vi "Connect.vi"(8 "error in (no error)":errorcluster caption="에러 입력(에러 없음)", 9 "원격 포트 또는 서비스 이름":u16, 10 "주소":string, 11 "RF Filter Box 입력":refnum<class "RF Filter Box.lvclass">) -> (0 "error out":errorcluster caption="에러 출력", 2 "Connected?":bool, 3 "RF Filter Box 출력":refnum<class "RF Filter Box.lvclass">)   [LabVIEW 2023, in "RF Switch Box.lvlib" / "RF Filter Box.lvclass"]
uses:
  RF Filter Box.lvclass
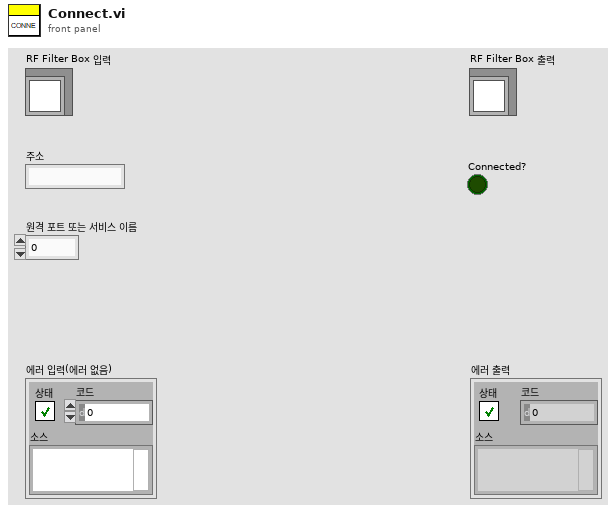
[diagram p1: front panel]
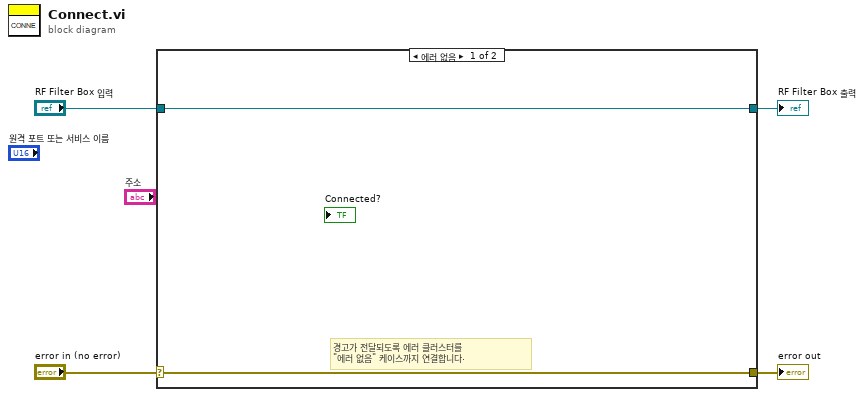
[diagram p0: block diagram]
diagram:
  n1 = case shown="에러 없음" "error in (no error)" {
    selector: "error in (no error)" -> [w5 w8]
    tunnel: [w5 w8] -> w3
    tunnel: [w6 w7] -> w1
    tunnel: "RF Filter Box 입력" -> [w6 w7]
    frame No Error {
      # "경고가 전달되도록 에러 클러스터를\n\"에러 없음\" 케이스까지 연결합니다."
    }
    frame Error {
    }
  }
  "error out" <- w3
  "RF Filter Box 출력" <- w1
